vi "Ball Valve labVIEW Code.vi"() -> ()   [LabVIEW 2025]
uses:
  PIDController/PIDController.lvclass
  spikeController/spikeController.lvclass
  labjacksModeEnum.ctl
  ControllerModeEnum.ctl
  modesEnum.ctl
  PIDController/PIDController.lvclass/PIDController.ctl
  0285ecf2-4d18-4427-ace1-61b1951a0741.vi
  d3b0afdc-d7ac-4f1a-8ecc-0aeb21fe1e80.vi
  0890acf7-df83-934e-a7ac-ae51bc85d557.vi
  d872897a-af24-4a4d-87bc-a1bb59a840a8.vi
  <vilib>/Instr/_visa.llb/VISA Configure Serial Port (Instr).vi
  PIDController/updateLastValues.vi
  <vilib>/Utility/file.llb/Write Delimited Spreadsheet (string).vi
  <vilib>/Utility/file.llb/Write Delimited Spreadsheet (DBL).vi
  <vilib>/ptbypt/NI_PtbyPt.lvlib
panel:
  out "arduino read response":string
  out "start time":u32
  in  "timeout":dbl=300.0
  in  "direction":i32=1
  in  "bias":dbl=100.0
  out "auto state":i32
  out "auto \ncycle_count":i32
  out "elements":T1[](array[typedef])
  out "Current Sensor Mode":T1=enum."Connect to Labjack"
  out "Labjack Handle":i32
  in  "Sensor Mode":enum16{"Fake", "Redboard", "Labjacks"}(ring)
  in  "Connect arduino":bool
  out "Connected":bool
  out "Set Angle":cluster{"Value":dbl, "Value":dbl}(graph)
  out "Read angle":dbl
  out "Target Angle":dbl
  out "arduino status":bool
  out "Motor Response":string
  in  "Disconnect":bool
  in  "Start Program":bool
  in  "Use Dummy Data":bool
  out "Pressure Sensor (integrated)":dbl(graph)
  out "PID Raw (one-by-one)":dbl(graph)
  out "target PID point":dbl
  out "auto k_d":dbl
  out "auto k_i":dbl
  out "auto k_p":dbl
  out "Array-to-save":dbl[][](array[numeric])
  out "to save":path
  out "Time Elapsed":dbl
  out "cycles_run":i32
  out "Autotune":bool
  in  "dt":dbl=0.1
  in  "tuning_rule":i32=3
  in  "min_cycles":i32=4
  in  "hysteresis":dbl=0.5
  in  "relay_amplitude":dbl=10.0
  in  "Exit Autotune":bool
  in  "Start AutoTune":bool
  out "last error":dbl
  in  "Use D1":bool
  in  "Use D2":bool
  in  "Use Avg":bool
  in  "Save Graphs":bool
  in  "Set setPoint":dbl=100.0 format="%.3f"
  in  "Set Angle":dbl format="%.3f"
  in  "setPoint Dial":dbl(knob) scale=0.0..1000.0
  in  "A_max":dbl=180.0
  in  "A_min":dbl
  in  "k_i":dbl
  in  "k_d":dbl
  in  "k_p":dbl
  out "SafetyClose":bool
  out "PID":bool
  out "Manual":bool
  out "Idle":bool
  out "Ducer1":bool
  out "Ducer2":bool
  out "Avg Ducers":bool
  out "Read Pressure Ducer":dbl
  out "Pressure Ducer 2":dbl
  in  "spikeController.lvclass":refnum<class "spikeController.lvclass">
  out "underAmin":bool
  out "overAmax":bool
  out "PID Raw Output":dbl[](graph)
  out "PID Translated Output":dbl
  out "PID Raw Output":dbl
  in  "loop stop 2":bool
  in  "loop stop 1":bool
  in  "PIDController.lvclass":refnum<class "PIDController.lvclass">
  in  "?":u32(colorbox)=16777225
  out "Pressure Sensor":dbl[](graph)
  in  "motor rpm indicator":dbl
  out "Motor Signal":string
  in  "stop program":bool
  in  "return spike":bool
  out "Position (measured)":dbl[](graph)
  out "Arduino Error":errorcluster
  in  "VISA resource Port":refnum<visa-resource-name>
  out "distance to go":dbl caption="Rotations to Go (º)" format="%.3f"
  out "Current Angle":dbl format="%.3f"
  in  "Set Angle (º)":dbl(slide) scale=0.1..180.0
  out "?":dbl(slide) scale=0.0..1000.0
  out "Stagnation Flow Temp (K)":dbl
  out "Pressure Ducer":dbl
  in  "Sensor Offsets":dbl[](array[numeric])=[10.0, 10.0, 0.0, 22.0]
  in  "Sensor K-values":dbl[](array[numeric])=[10.0, 10.0, 0.0, 22.0]
  in  "Exit PID Mode":bool
  in  "manual exit button":bool
  in  "Motor Control Loop Rate (ms)":dbl
  out "Set Motor RPM":dbl(knob) scale=0.0..200.0
  in  "PID Mode":bool
  in  "Manual Positioning Mode":bool
  in  "Stop Sensors":bool
  in  "Sensor Loop Rate (ms)":dbl
  out "Time Since Start (s)\n(For Reference Only)":dbl format="%.2f"
  in  "Start Sensors":bool
  in  "Load Inputs":bool
  in  "Save Inputs":bool
  out "Port":i32
  out "ConnectionType":i32
  out "DeviceType":i32
  out "Labjack error":errorcluster
  # "(dial indicator for range)"
  # "34HS59-6004S Motor Torque Curve (For Reference)"
  # "Labjack/Arduino Resources"
  # "Inputs and LabJack Sensor Monitors"
  # "PID Inputs"
  # "Motor RPM >200 RPM"
  # "Potentiometer"
  # "Inefficent Torque for High Mass Flow/Thrust Tests"
  # "Ducer"
  # "<-- Uses same setpoint"
  # "Thermocouple"
  # "Motor RPM < 200 RPM"
  # "COM Port for Arduino"
  # "Ball valve"
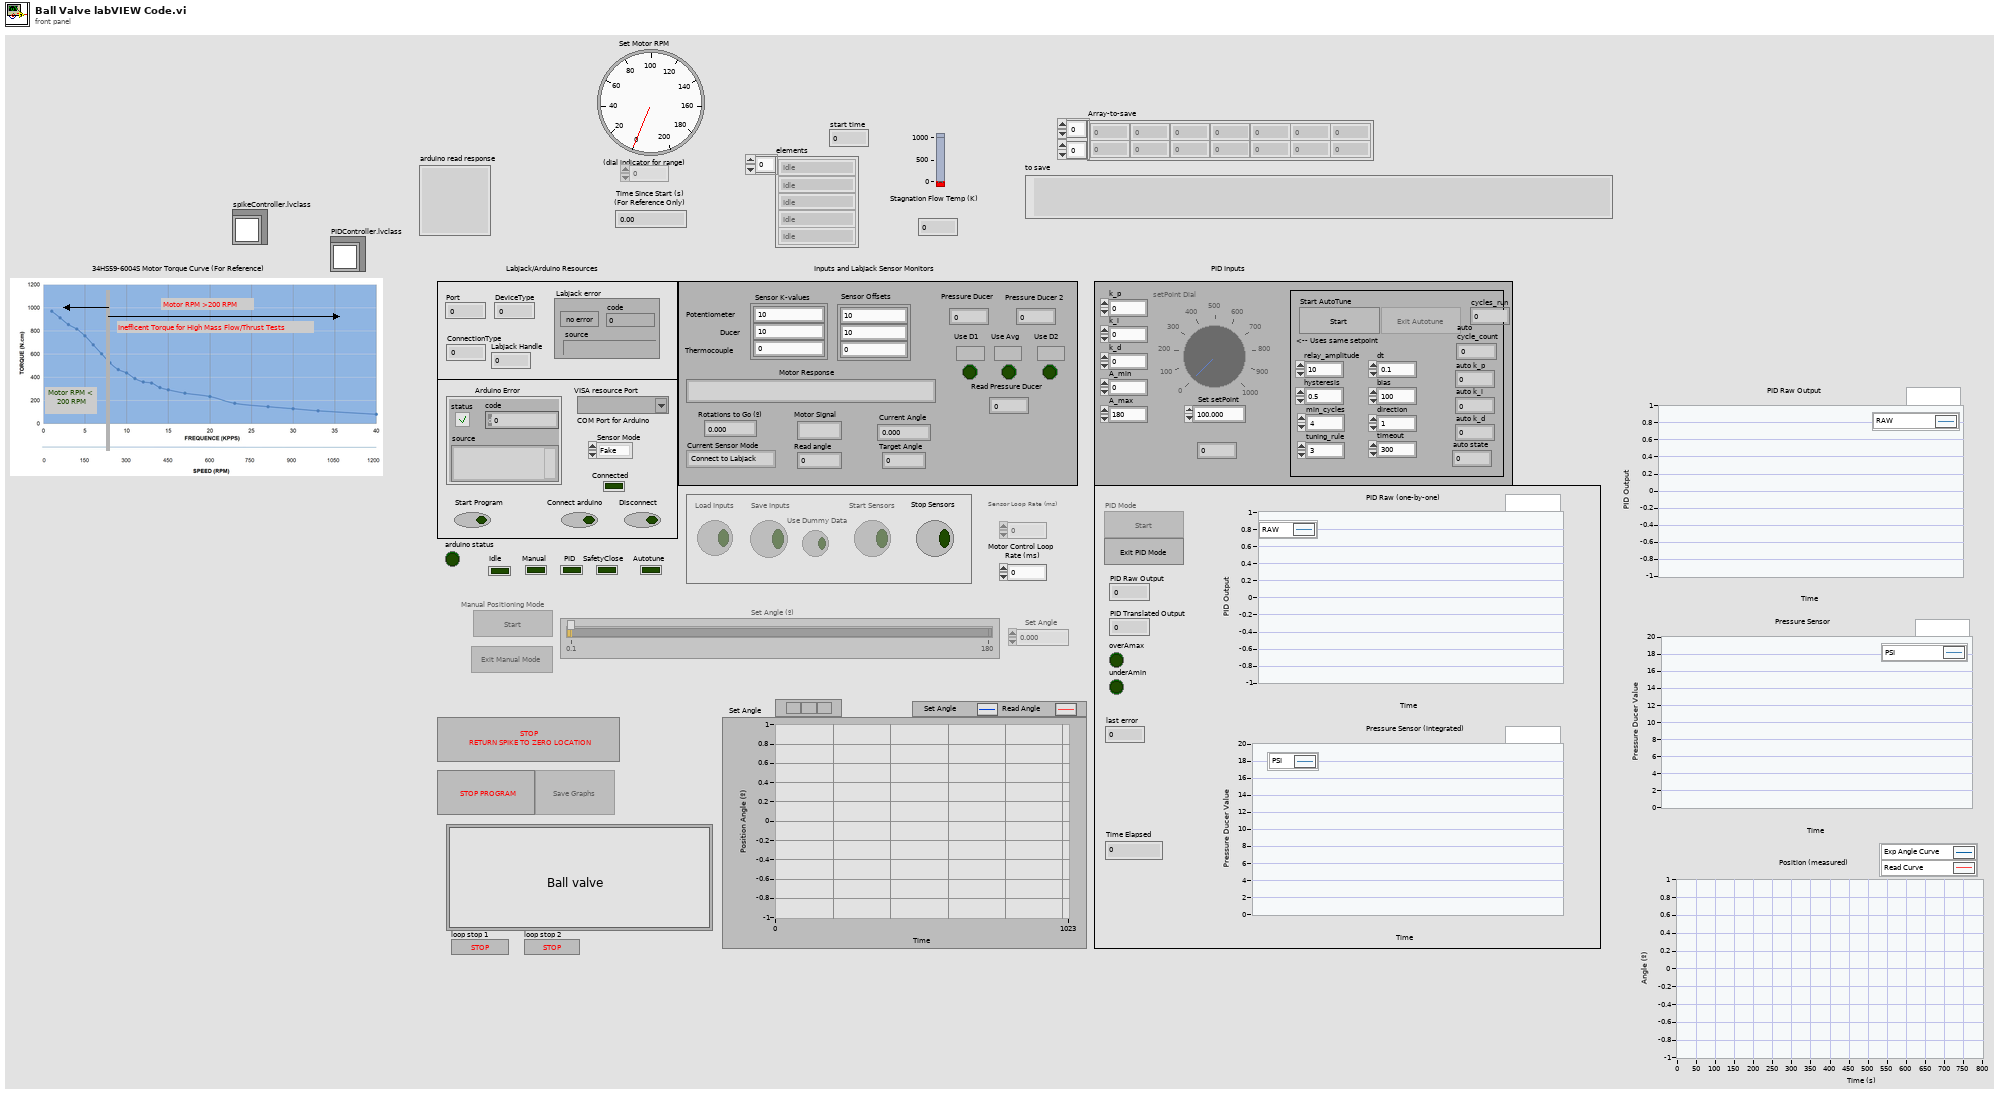
[diagram p1: front panel]
types:
  T1 = typedef "labjacksModeEnum.ctl" = enum16{"Idle", "Connect to Labjack", "Start sensors", "Dummy data", "Arduino Sensors", "load values"}
  T2 = typedef "ControllerModeEnum.ctl" = enum16{"", "startControllers", "IdleControllers"}
  T3 = typedef "modesEnum.ctl" = enum16{"relay_autotune", "SafetyOpen", "SafetyClose", "SaveFile", "PIDControl", "ManualControl", "Idle"}
  T4 = enum16{"Potentiometer", "Ducer", "Thermocouple", "Ducer2"}
  T5 = enum16{"Ducer", "Ducer2", "Thermocouple", "Potentiometer"}
  T6 = enum8{"Enabled", "Disabled", "Disabled and Grayed Out"}
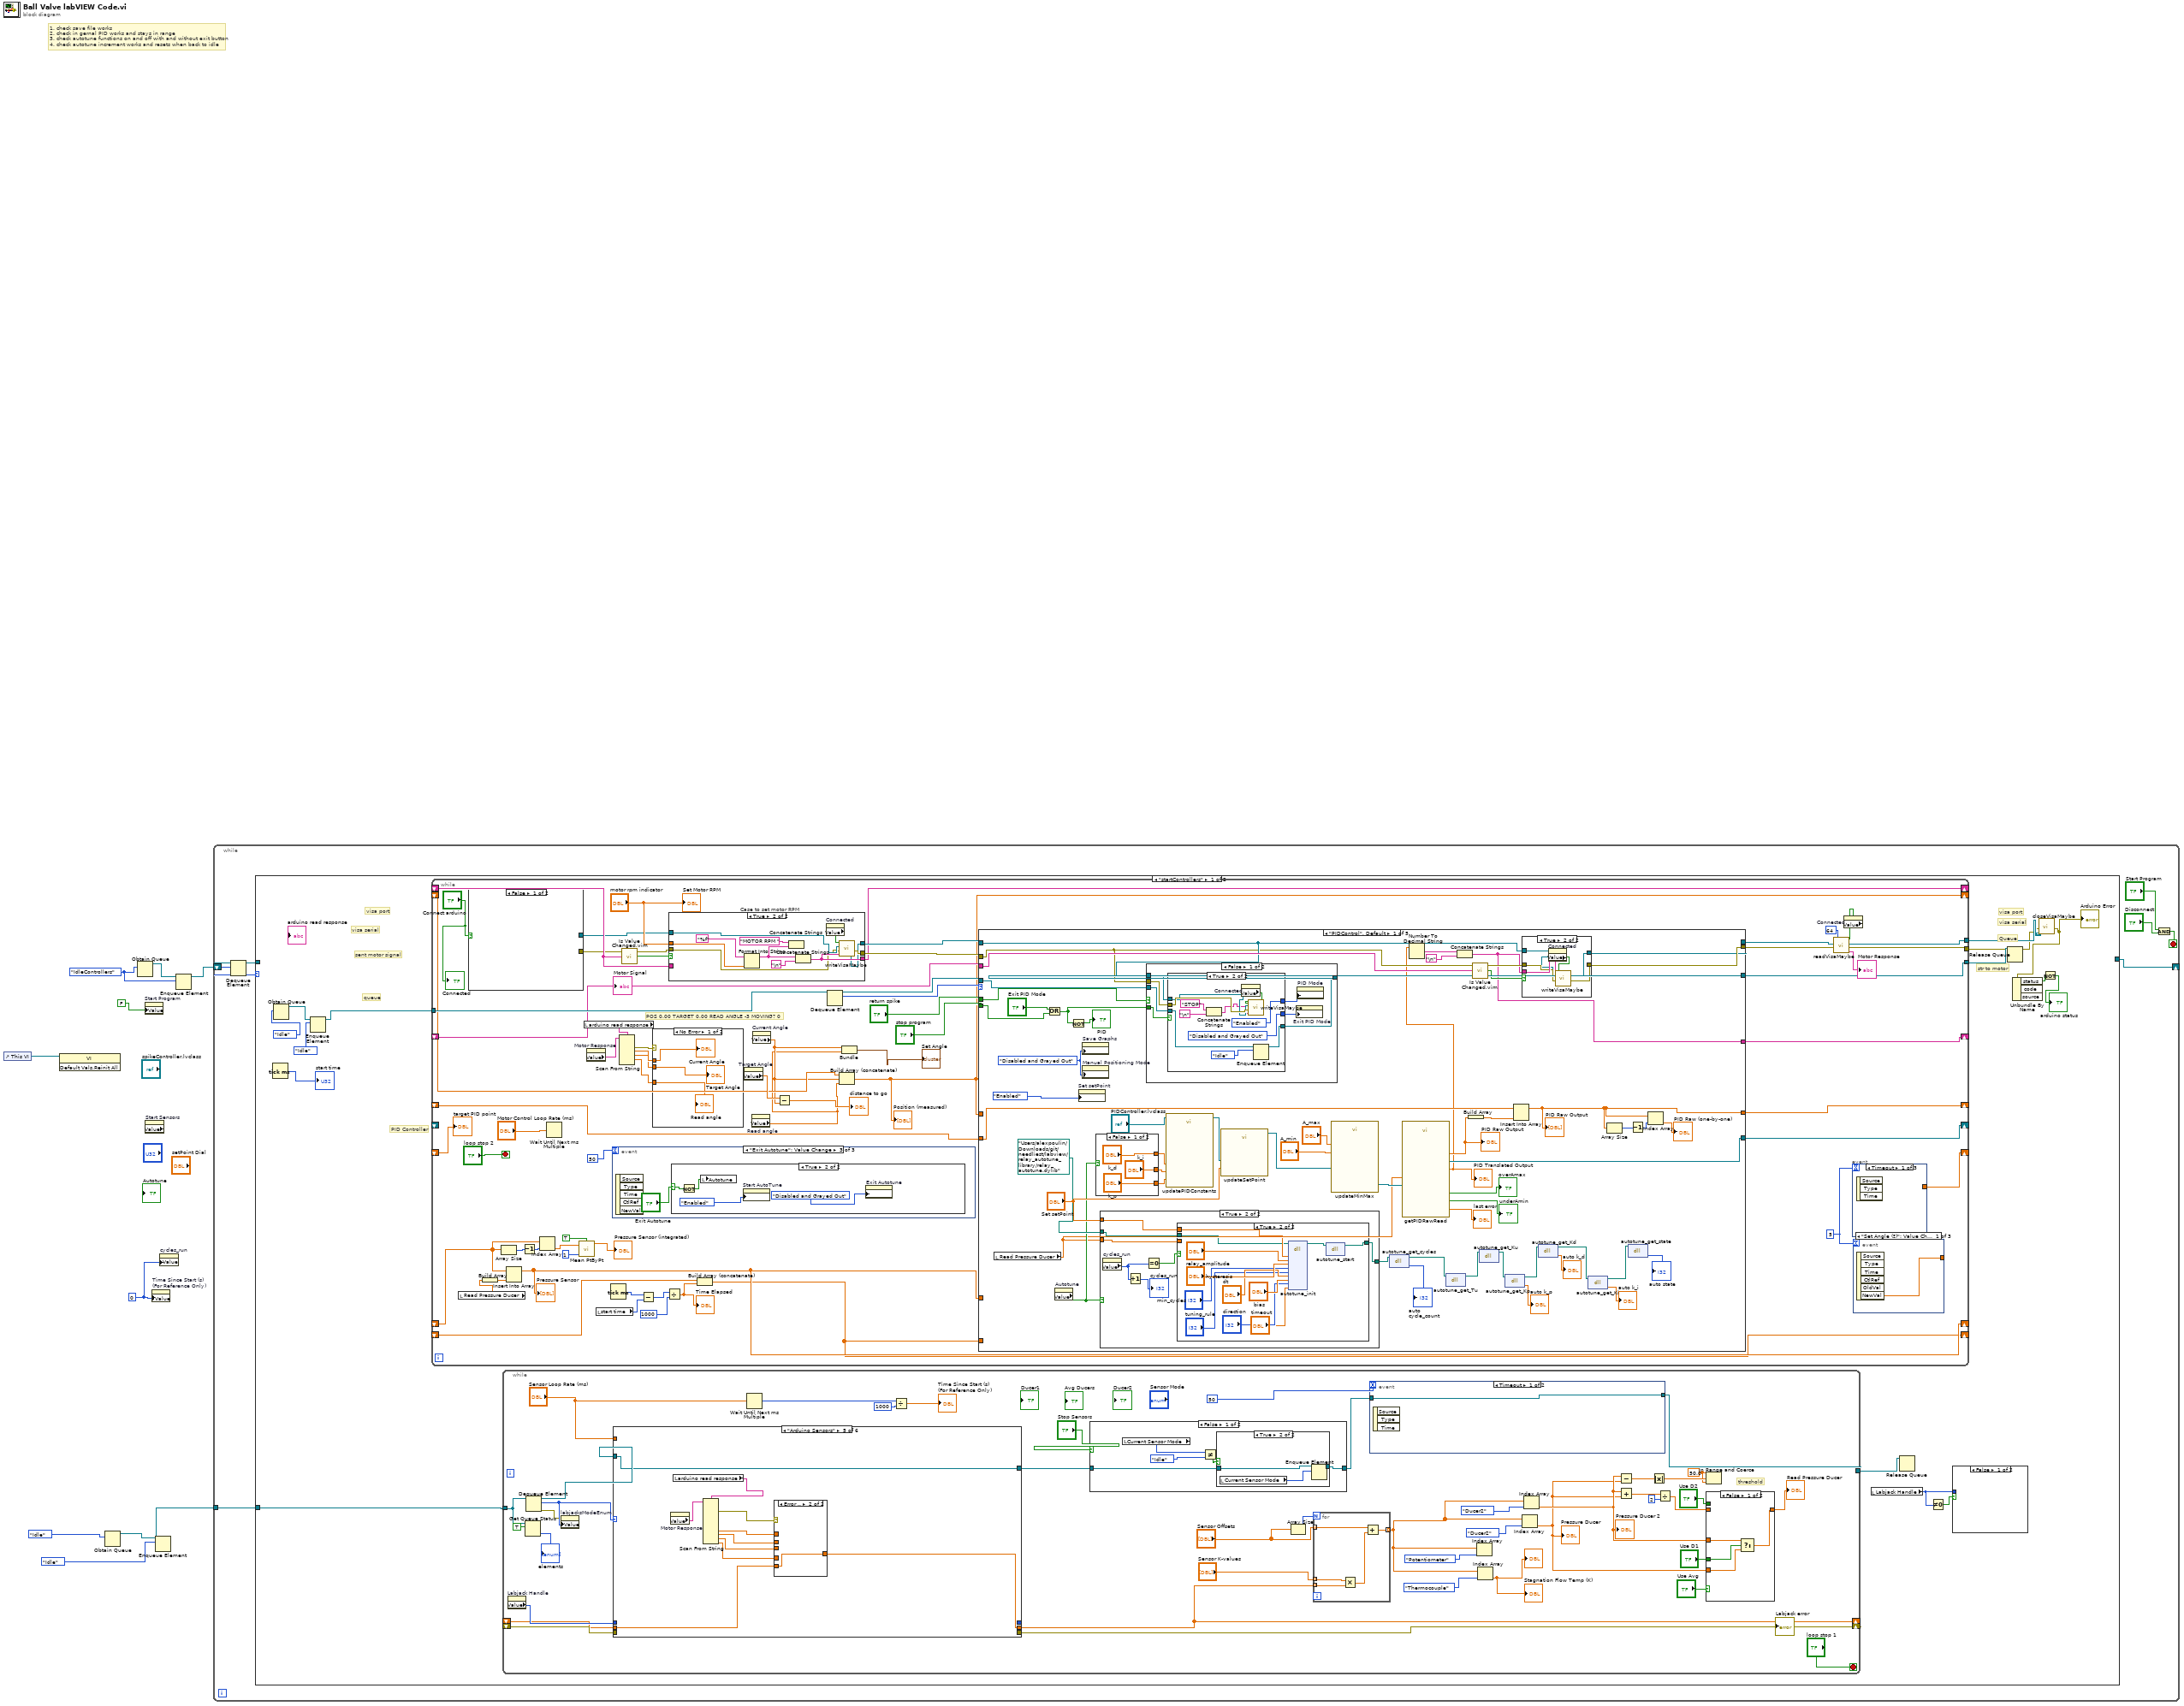
[diagram p0: block diagram]
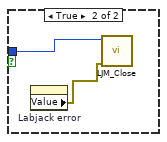
[diagram p2: hidden frame]
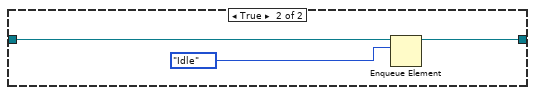
[diagram p4: hidden frame]
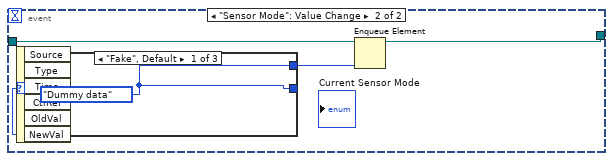
[diagram p5: hidden frame]
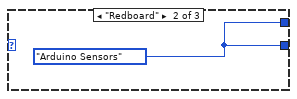
[diagram p6: hidden frame]
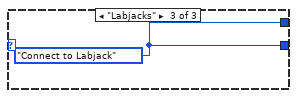
[diagram p7: hidden frame]
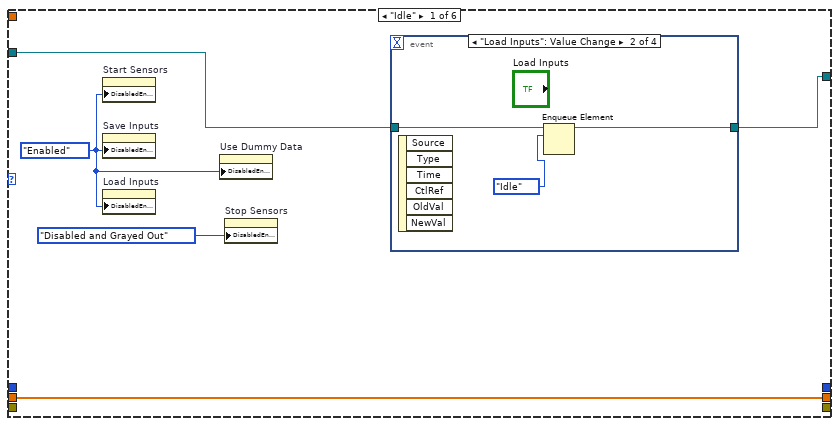
[diagram p9: hidden frame]
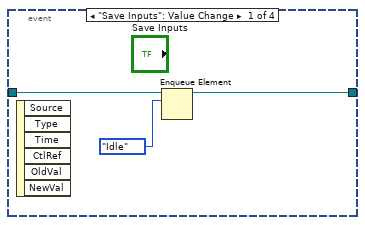
[diagram p10: hidden frame]
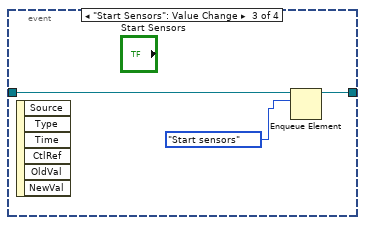
[diagram p11: hidden frame]
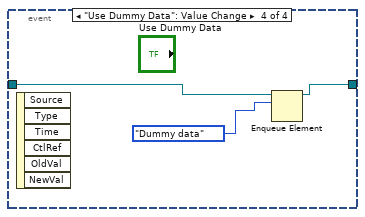
[diagram p12: hidden frame]
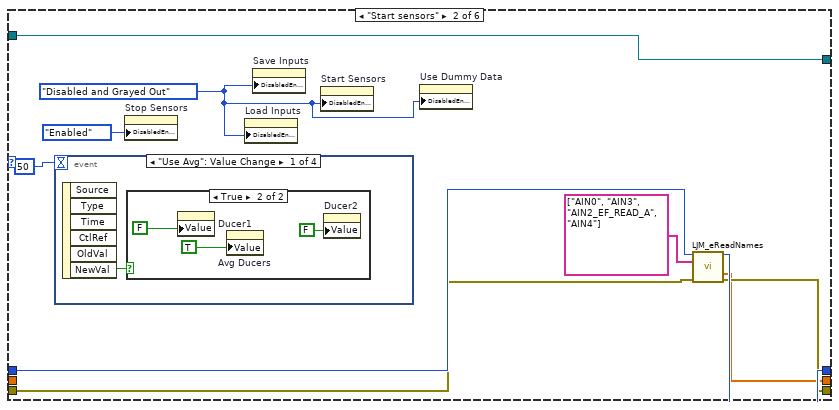
[diagram p13: hidden frame]
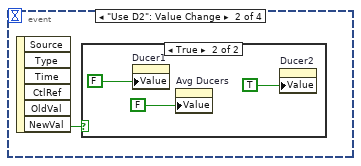
[diagram p15: hidden frame]
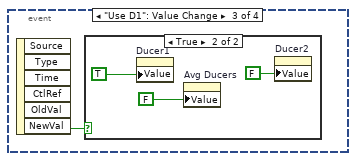
[diagram p17: hidden frame]
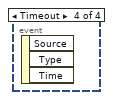
[diagram p19: hidden frame]
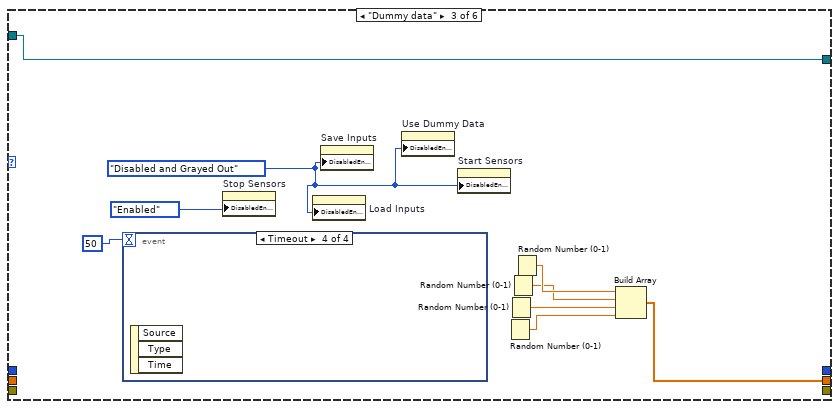
[diagram p20: hidden frame]
diagram:
  w2 = u32 0 ("Time Since Start (s)\n(For Reference Only) 2")
  w9 = ControllerModeEnum."IdleControllers" ("ControllerModeEnum")
  # "1. check save file works\n2. check in gernal PID works and stays in range\n3. check autotune functions on and off with and without exit button\n4. check autotune increment works and resets when back to idle"
  n1 = control-ref of="This VI"() -> (w1:refnum<vi>)
  n2 = invoke class="VI" method="Default Vals.Reinit All"(reference=w1) -> ()  [unwired: 2 in, 3 out]
  n3 = Obtain Queue(element data type=labjacksModeEnum."Idle" ("labjacksModeEnum")) -> (queue out=w5:refnum<queue>)  [unwired: 4 in, 2 out]
  n4 = Obtain Queue(element data type=w9) -> (queue out=w10:refnum<queue>)  [unwired: 4 in, 2 out]
  n5 = property on="Start Program" class="Bool (strict)"("Value"=FALSE) -> ()  [unwired: 2 in, 2 out]
  n6 = property on="Start Sensors" class="Bool" props=["Value"]() -> ()  [unwired: 2 in, 3 out]
  n7 = property on="Time Since Start (s)\n(For Reference Only)" class="DigNum (strict)"("Value"=w2) -> ()  [unwired: 2 in, 2 out]
  n8 = Enqueue Element(queue=w5, element=labjacksModeEnum."Idle" ("labjacksModeEnum")) -> (queue out=w3:refnum<queue>)  [unwired: 2 in, 2 out]
  n9 = property on="cycles_run" class="DigNum (strict)"("Value"=w2) -> ()  [unwired: 2 in, 2 out]
  n10 = Enqueue Element(queue=w10, element=w9) -> (queue out=w8:refnum<queue>)  [unwired: 2 in, 2 out]
  n11 = while {
    shift-right: [w14] -> _
    shift-left: w8 -> [w12]
    tunnel: w3 -> [w11]
    stop <- w16 stop-if-true
    n12 = Dequeue Element(queue=w12) -> (queue out=w13:refnum<queue>, element=w15:T2)  [unwired: 2 in, 2 out]
    n13 = case shown="\"startControllers\"" w15 {
      tunnel: [_ w568] -> w14
      tunnel: w13 -> [_ w567]
      tunnel: w11 -> [w22 _]
      frame "startControllers" {
        # "str to motor"
        # "Queue"
        # "sent motor signal"
        # "PID Controller"
        # "visa serial"
        # "visa port"
        # "queue"
        # "visa port"
        # "visa serial"
        n14 = Tick Count (ms)() -> (millisecond timer value=→"start time":u32)
        n15 = Obtain Queue(element data type=modesEnum."Idle" ("modesEnum")) -> (queue out=w33:refnum<queue>)  [unwired: 4 in, 2 out]
        n16 = Enqueue Element(queue=w33, element=modesEnum."Idle" ("modesEnum")) -> (queue out=w32:refnum<queue>)  [unwired: 2 in, 2 out]
        n17 = while {
          tunnel: w32 -> [w260]
          tunnel: [w258] -> w31
          tunnel: [w220] -> w26
          tunnel: [w221] -> w25
          shift-right: [w256] -> _
          shift-left: _ -> [w255]
          shift-right: [w251] -> _
          shift-left: _ -> [w250]
          shift-right: [w247] -> _
          shift-left: _ -> [_]
          shift-right: [w200] -> _
          shift-left: _ -> [w202]
          shift-right: [w244] -> _
          shift-left: _ -> [w245]
          shift-right: [w228] -> _
          shift-left: _ -> [w232]
          shift-right: [w240] -> _
          shift-left: _ -> [w241]
          shift-right: [w199] -> _
          shift-left: _ -> [w211]
          stop <- "loop stop 2" stop-if-true
          w239 = 5
          # "POS 0.00 TARGET 0.00 READ ANGLE -3 MOVING? 0"
          n18 = local read "Read Pressure Ducer"() -> (w201:dbl)
          n19 = case shown="False" "Connect arduino" {
            tunnel: [_ w271] -> w219
            tunnel: [_ w270] -> w218
            frame False {
            }
            frame True {
              w272 = u16 0 items=["None", "XON/XOFF", "RTS/CTS", "XON/XOFF & RTS/CTS", "DTR/DSR", "XON/XOFF & DTR/DSR"] ("flow control (0:none)")
              w273 = u16 10 items=["1.0"=10, "1.5"=15, "2.0"=20] ("stop bits (10: 1 bit)")
              n20 = call-poly "VISA Configure Serial Port"("VISA resource name"="VISA resource Port", "Enable Termination\nChar (T)"=TRUE ("Enable Termination\nChar (T)"), "baud rate (9600)"=u32 115200, "data bits (8)"=u16 8, "parity (0:none)"=enum16{"None", "Odd", "Even", "Mark", "Space"}."None", "stop bits (10: 1 bit)"=w273, "flow control (0:none)"=w272) -> ("VISA resource name out"=w271:refnum<visa-resource-name>, "error out"=w270:errorcluster)  [unwired: 7 in]
            }
          }
          n21 = Build Array(w201) -> (w205:dbl[])
          n22 = Array Size(array=w202) -> (size(s)=w208:i32)
          n23 = Insert Into Array(array=w202, new element=w205) -> (w200:dbl[])  [unwired: 1 in]
          "Pressure Sensor" <- w200
          n24 = Decrement(x=w208) -> (x-1=w209:i32)
          n25 = Index Array(array=w202, index=w209) -> (element=w206:dbl)
          n26 = Wait Until Next ms Multiple(millisecond multiple="Motor Control Loop Rate (ms)") -> ()  [unwired: 1 out]
          n27 = call <vilib>:"Mean PtByPt.vi"("x"=w206, "sample length"=1, "initialize"=TRUE) -> ("mean"=→"Pressure Sensor (integrated)":dbl)  [unwired: 1 in, 1 out]
          n28 = local read "arduino read response"() -> (w198:string)
          n29 = property on="Motor Response" class="Str"() -> ("Value"=w238:string)  [unwired: 2 in, 2 out]
          n30 = local read "start time"() -> (w215:u32)
          n31 = Tick Count (ms)() -> (millisecond timer value=w212:u32)
          n32 = event shown="[2] \"Exit Autotune\": Value Change" {
            selector: _ -> [_ _ _]
            dyn-events: _ -> [_ _ _]
            timeout: 50 -> [_ _ _]
            event Timeout {
              n33 = event-data() -> ()  [unwired: 1 in, 3 out]
            }
            event "Start AutoTune": Value Change {
              n34 = event-data() -> ()  [unwired: 1 in, 5 out]
              n35 = case shown="True" "Start AutoTune" {
                selector: "Start AutoTune" -> [w264 _]
                frame True {
                  n36 = local write "Autotune"(w264) -> ()
                  n37 = property on="Exit Autotune" class="Bool"("DisabledEnum"=T6."Enabled" ("Disabled")) -> ()  [unwired: 2 in, 2 out]
                  n38 = property on="Start AutoTune" class="Bool"("DisabledEnum"=T6."Disabled and Grayed Out" ("Disabled")) -> ()  [unwired: 2 in, 2 out]
                }
                frame False {
                }
              }
            }
            event "Exit Autotune": Value Change {
              n39 = event-data() -> ()  [unwired: 1 in, 5 out]
              n40 = case shown="True" "Exit Autotune" {
                selector: "Exit Autotune" -> [_ w269]
                frame False {
                }
                frame True {
                  n41 = Not(x=w269) -> (.not. x?=w266:bool)
                  n42 = local write "Autotune"(w266) -> ()
                  n43 = property on="Start AutoTune" class="Bool"("DisabledEnum"=T6."Enabled" ("Disabled")) -> ()  [unwired: 2 in, 2 out]
                  n44 = property on="Exit Autotune" class="Bool"("DisabledEnum"=T6."Disabled and Grayed Out" ("Disabled")) -> ()  [unwired: 2 in, 2 out]
                }
              }
            }
          }
          n45 = Scan From String(format string=w198, input string=w238) -> (error out=w237:errorcluster, output 1=w236:dbl, output 2=w234:dbl, output 3=w231:dbl)  [unwired: 7 in, 2 out]
          n46 = call "Is Value Changed.vim"("value"=w250) -> ("changed or first call?"=w252:bool)
          n47 = Subtract(x=w212, y=w215) -> (x-y=w214:u32)
          n48 = case shown="No Error" w237 {
            tunnel: w236 -> [w280 _]
            tunnel: w234 -> [w281 _]
            tunnel: w231 -> [w279 _]
            frame No Error {
              "Target Angle" <- w281
              "Current Angle" <- w280
              "Read angle" <- w279
            }
            frame Error {
            }
          }
          n49 = Divide(x=w214, y=1000) -> (x/y=w210:dbl)
          "Time Elapsed" <- w210
          n50 = case "Case to set motor RPM" shown="True" w252 {
            tunnel: w218 -> [w291 w296]
            tunnel: [w287 w298] -> w251
            tunnel: w219 -> [w292 w297]
            tunnel: [w291 w295] -> w254
            tunnel: [w292 w294] -> w253
            tunnel: "motor rpm indicator" -> [w290 w303]
            tunnel: w250 -> [_ _]
            frame False {
              n51 = Format Into String(format string="%f", w290) -> (resulting string=w288:string)  [unwired: 2 in, 1 out]
              n52 = Concatenate Strings(w288, "\n" ("string")) -> (w287:string)
            }
            frame True {
              n53 = Format Into String(format string="%f", w303) -> (resulting string=w301:string)  [unwired: 2 in, 1 out]
              n54 = Concatenate Strings("MOTOR RPM " ("format string"), w301) -> ()  [unwired: 1 out]
              n55 = Concatenate Strings(w301, "\n") -> (w298:string)
              n56 = property on="Connected" class="Bool (strict)"() -> ("Value"=w293:bool)  [unwired: 2 in, 2 out]
              n57 = call "writeVisaMaybe.vi"("String to Write"=w298, "error in"=w296, "VISA resource name in"=w297, "VISA connected?"=w293) -> ("error out"=w295:errorcluster, "VISA resource name out"=w294:refnum<visa-resource-name>)  [unwired: 2 in]
            }
          }
          n58 = Build Array (concatenate)(w211, w210) -> (w199:dbl[])
          n59 = property on="Target Angle" class="DigNum (strict)"() -> ("Value"=w233:dbl)  [unwired: 2 in, 2 out]
          n60 = property on="Read angle" class="DigNum (strict)"() -> ("Value"=w229:dbl)  [unwired: 2 in, 2 out]
          n61 = property on="Current Angle" class="DigNum (strict)"() -> ("Value"=w230:dbl)  [unwired: 2 in, 2 out]
          n62 = Subtract(x=w233, y=w230) -> (x-y=→"distance to go":dbl)
          n63 = Dequeue Element(queue=w260) -> (queue out=w242:refnum<queue>, element=w259:T3)  [unwired: 2 in, 2 out]
          n64 = Build Array (concatenate)(w232, w230, w229) -> (w228:dbl[])
          "Position (measured)" <- w228
          n65 = Bundle("Value"=w230, "Value"=w229) -> (→"Set Angle":cluster{"Value":dbl, "Value":dbl})  [unwired: 1 in]
          n66 = case shown="\"PIDControl\", Default" w259 {
            tunnel: [w351 w436 w473 w506 _] -> w258
            tunnel: w242 -> [w327 w432 w474 w505 _]
            tunnel: w253 -> [w326 w423 w471 w509 _]
            tunnel: [w315 w422 w470 w501 _] -> w226
            tunnel: w254 -> [w314 w425 w469 w510 _]
            tunnel: [w316 w421 w468 w507 _] -> w224
            tunnel: [w313 w424 w478 w508 _] -> w256
            tunnel: w255 -> [w347 _ w478 w504 _]
            tunnel: "return spike" -> [w350 w437 _ _ _]
            tunnel: [w358 _ _ _ _] -> w247
            tunnel: w245 -> [w320 _ _ _ w551]
            tunnel: [w312 _ _ _ _] -> w244
            tunnel: "stop program" -> [w352 w428 _ _ _]
            tunnel: w228 -> [_ _ _ _ w553]
            tunnel: w200 -> [_ _ _ _ w550]
            tunnel: w199 -> [_ _ _ _ w552]
            frame "PIDControl", Default {
              w330 = T6."Disabled and Grayed Out" ("Disabled")
              n67 = local read "Read Pressure Ducer"() -> (w304:dbl)
              n68 = Or(x="Exit PID Mode", y=w352) -> (x .or. y?=w328:bool)
              n69 = property on="Autotune" class="Bool (strict)"() -> ("Value"=w305:bool)  [unwired: 2 in, 2 out]
              n70 = Not(x=w328) -> (.not. x?=→"PID":bool)
              n71 = property on="Set setPoint" class="DigNum (strict)"("DisabledEnum"=T6."Enabled" ("Disabled")) -> ()  [unwired: 2 in, 2 out]
              n72 = property on="Save Graphs" class="Bool"("DisabledEnum"=w330) -> ()  [unwired: 2 in, 2 out]
              n73 = property on="Manual Positioning Mode" class="Bool"("DisabledEnum"=w330) -> ()  [unwired: 2 in, 2 out]
              n74 = case shown="False" w305 {
                tunnel: ["k_p" w362] -> w339
                tunnel: ["k_i" w363] -> w338
                tunnel: ["k_d" w364] -> w337
                frame False {
                }
                frame True {
                  n75 = local read "auto k_i"() -> (w363:dbl)
                  n76 = local read "auto k_d"() -> (w364:dbl)
                  n77 = local read "auto k_p"() -> (w362:dbl)
                }
              }
              n78 = case shown="True" w305 {
                tunnel: path "/Users/alexpoulin/Downloads/git/needliest/labview/relay_autotune_library/relay_autotune.dylib" -> [w371 w376]
                tunnel: [w371 w375] -> w340
                tunnel: w304 -> [_ w374]
                tunnel: "Set setPoint" -> [_ w372]
                frame False {
                }
                frame True {
                  n79 = property on="cycles_run" class="DigNum (strict)"() -> ("Value"=w378:i32)  [unwired: 2 in, 2 out]
                  n80 = Increment(x=w378) -> (x+1=→"cycles_run":i32)
                  n81 = Equal To 0?(x=w378) -> (x = 0?=w373:bool)
                  n82 = case shown="True" w373 {
                    tunnel: w376 -> [w381 w385]
                    tunnel: [w380 w392] -> w375
                    tunnel: w374 -> [w379 _]
                    tunnel: w372 -> [_ w386]
                    frame False {
                      n83 = dll-call lib="Users/alexpoulin/Downloads/git/needliest/labview/relay_autotune_library/relay_autotune.dylib" fn="autotune_update"(path in=w381, "pv"=w379) -> (path out=w380:path)  [unwired: 4 in, 1 out]
                    }
                    frame True {
                      n84 = dll-call lib="Users/alexpoulin/Downloads/git/needliest/labview/relay_autotune_library/relay_autotune.dylib" fn="autotune_init"(path in=w385, "setpoint"=w386, "relay_amplitude"="relay_amplitude", "hysteresis"="hysteresis", "min_cycles"="min_cycles", "tuning_rule"="tuning_rule", "dt"="dt", "bias"="bias", "direction"="direction", "timeout"="timeout") -> (path out=w393:path)  [unwired: 12 in, 1 out]
                      n85 = dll-call lib="Users/alexpoulin/Downloads/git/needliest/labview/relay_autotune_library/relay_autotune.dylib" fn="autotune_start"(path in=w393) -> (path out=w392:path)  [unwired: 3 in, 1 out]
                    }
                  }
                }
              }
              n86 = case shown="False" w350 {
                tunnel: [w396 w419] -> w351
                tunnel: w328 -> [w400 _]
                tunnel: w327 -> [w399 w417]
                tunnel: w326 -> [w398 _]
                tunnel: w314 -> [w397 _]
                frame False {
                  n87 = case shown="True" w400 {
                    tunnel: w399 -> [w405 w416]
                    tunnel: [w404 w415] -> w396
                    tunnel: w398 -> [_ w407]
                    tunnel: w397 -> [_ w408]
                    tunnel: [T6."Disabled and Grayed Out" ("Disabled") T6."Enabled" ("Disabled")] -> w395
                    tunnel: [T6."Enabled" ("Disabled") T6."Disabled and Grayed Out" ("Disabled")] -> w394
                    frame False {
                      n88 = Enqueue Element(queue=w405, element=modesEnum."PIDControl" ("modesEnum")) -> (queue out=w404:refnum<queue>)  [unwired: 2 in, 2 out]
                    }
                    frame True {
                      n89 = Concatenate Strings("STOP" ("write buffer"), "\n" ("write buffer")) -> (w406:string)
                      n90 = property on="Connected" class="Bool (strict)"() -> ("Value"=w409:bool)  [unwired: 2 in, 2 out]
                      n91 = call "writeVisaMaybe.vi"("String to Write"=w406, "error in"=w408, "VISA resource name in"=w407, "VISA connected?"=w409) -> ()  [unwired: 2 in, 2 out]
                      n92 = Enqueue Element(queue=w416, element=modesEnum."Idle" ("modesEnum")) -> (queue out=w415:refnum<queue>)  [unwired: 2 in, 2 out]
                    }
                  }
                  n93 = property on="Exit PID Mode" class="Bool"("DisabledEnum"=w394) -> ()  [unwired: 2 in, 2 out]
                  n94 = property on="PID Mode" class="Bool"("DisabledEnum"=w395) -> ()  [unwired: 2 in, 2 out]
                }
                frame True {
                  n95 = Enqueue Element(queue=w417, element=modesEnum."SafetyClose" ("modesEnum")) -> (queue out=w419:refnum<queue>)  [unwired: 2 in, 2 out]
                }
              }
              n96 = call "updatePIDConstants.vi"("new k_d"=w337, "new k_p"=w339, "new k_i"=w338, "PIDController in"="PIDController.lvclass") -> ("PIDController out"=w333:refnum<class "PIDController.lvclass">)  [unwired: 6 in, 1 out]
              n97 = call "updateSetPoint.vi"("new setpoint"="Set setPoint", "PIDController in"=w333) -> ("PIDController out"=w332:refnum<class "PIDController.lvclass">)  [unwired: 8 in, 1 out]
              n98 = call "updateMinMax.vi"("a_max"="A_max", "a_min"="A_min", "PIDController in"=w332) -> ("PIDController out"=w331:refnum<class "PIDController.lvclass">)  [unwired: 7 in, 1 out]
              n99 = dll-call lib="Users/alexpoulin/Downloads/git/needliest/labview/relay_autotune_library/relay_autotune.dylib" fn="autotune_get_cycles"(path in=w340) -> (path out=w346:path, "g_ctx.cycle_count"=→"auto \ncycle_count":i32)  [unwired: 2 in, 1 out]
              n100 = call "getPIDRawRead.vi"("sensorValue"=w304, "PIDController in"=w331) -> ("overAmin"=→"underAmin":bool, "translatedPIDOutput"=w309:dbl, "PIDRawRead"=w357:dbl, "PIDController out"=w358:refnum<class "PIDController.lvclass">, "underAmax"=→"overAmax":bool, "lastErrorRead"=→"last error":dbl)  [unwired: 4 in]
              "PID Raw Output" <- w357
              "PID Translated Output" <- w309
              n101 = Number To Decimal String(number=w309) -> (decimal integer string=w310:string)  [unwired: 1 in]
              n102 = dll-call lib="Users/alexpoulin/Downloads/git/needliest/labview/relay_autotune_library/relay_autotune.dylib" fn="autotune_get_Tu"(path in=w346) -> (path out=w345:path)  [unwired: 3 in, 1 out]
              n103 = Concatenate Strings(w310, "\n") -> (w313:string)
              n104 = Build Array(w357) -> (w356:dbl[])
              n105 = call "Is Value Changed.vim"("value"=w347) -> ("changed or first call?"=w317:bool)
              n106 = dll-call lib="Users/alexpoulin/Downloads/git/needliest/labview/relay_autotune_library/relay_autotune.dylib" fn="autotune_get_Ku"(path in=w345) -> (path out=w344:path)  [unwired: 3 in, 1 out]
              n107 = dll-call lib="Users/alexpoulin/Downloads/git/needliest/labview/relay_autotune_library/relay_autotune.dylib" fn="autotune_get_Kp"(path in=w344) -> (path out=w343:path, "g_ctx.Kp"=→"auto k_p":dbl)  [unwired: 2 in, 1 out]
              n108 = Insert Into Array(array=w320, new element=w356) -> (w312:dbl[])  [unwired: 1 in]
              "PID Raw Output" <- w312
              n109 = case shown="True" w317 {
                tunnel: w314 -> [_ w369]
                tunnel: w326 -> [_ w368]
                tunnel: [_ w367] -> w316
                tunnel: [_ w366] -> w315
                tunnel: w313 -> [_ w370]
                frame False {
                }
                frame True {
                  n110 = property on="Connected" class="Bool (strict)"() -> ("Value"=w365:bool)  [unwired: 2 in, 2 out]
                  n111 = call "writeVisaMaybe.vi"("String to Write"=w370, "error in"=w369, "VISA resource name in"=w368, "VISA connected?"=w365) -> ("error out"=w367:errorcluster, "VISA resource name out"=w366:refnum<visa-resource-name>)  [unwired: 2 in]
                }
              }
              n112 = dll-call lib="Users/alexpoulin/Downloads/git/needliest/labview/relay_autotune_library/relay_autotune.dylib" fn="autotune_get_Kd"(path in=w343) -> (path out=w342:path, "g_ctx.Kd"=→"auto k_d":dbl)  [unwired: 2 in, 1 out]
              n113 = dll-call lib="Users/alexpoulin/Downloads/git/needliest/labview/relay_autotune_library/relay_autotune.dylib" fn="autotune_get_Ki"(path in=w342) -> (path out=w341:path, "g_ctx.Ki"=→"auto k_i":dbl)  [unwired: 2 in, 1 out]
              n114 = Array Size(array=w312) -> (size(s)=w319:i32)
              n115 = dll-call lib="Users/alexpoulin/Downloads/git/needliest/labview/relay_autotune_library/relay_autotune.dylib" fn="autotune_get_state"(path in=w341) -> ("g_ctx.state"=→"auto state":i32)  [unwired: 2 in, 2 out]
              n116 = Decrement(x=w319) -> (x-1=w318:i32)
              n117 = Index Array(array=w312, index=w318) -> (element=→"PID Raw (one-by-one)":dbl)
            }
            frame "ManualControl" {
              w431 = T6."Enabled" ("Disabled")
              w434 = T6."Disabled and Grayed Out" ("Disabled")
              n118 = Or(x=w428, y="manual exit button") -> (x .or. y?=w438:bool)
              n119 = Or(x=w437, y=w438) -> (x .or. y?=w433:bool)
              n120 = Not(x=w433) -> (.not. x?=→"Manual":bool)
              n121 = case shown="False" w437 {
                tunnel: [w441 w464] -> w436
                tunnel: w433 -> [w445 _]
                tunnel: w432 -> [w444 w462]
                tunnel: w423 -> [w443 _]
                tunnel: w425 -> [w442 _]
                frame False {
                  n122 = case shown="True" w445 {
                    tunnel: w444 -> [w450 w461]
                    tunnel: [w449 w460] -> w441
                    tunnel: w443 -> [_ w452]
                    tunnel: w442 -> [_ w453]
                    tunnel: [T6."Enabled" ("Disabled") T6."Disabled and Grayed Out" ("Disabled")] -> w440
                    tunnel: [T6."Disabled and Grayed Out" ("Disabled") T6."Enabled" ("Disabled")] -> w439
                    frame False {
                      n123 = Enqueue Element(queue=w450, element=modesEnum."ManualControl" ("modesEnum")) -> (queue out=w449:refnum<queue>)  [unwired: 2 in, 2 out]
                    }
                    frame True {
                      n124 = Concatenate Strings("STOP" ("write buffer"), "\n") -> (w451:string)
                      n125 = property on="Connected" class="Bool (strict)"() -> ("Value"=w454:bool)  [unwired: 2 in, 2 out]
                      n126 = call "writeVisaMaybe.vi"("String to Write"=w451, "error in"=w453, "VISA resource name in"=w452, "VISA connected?"=w454) -> ()  [unwired: 2 in, 2 out]
                      n127 = Enqueue Element(queue=w461, element=modesEnum."Idle" ("modesEnum")) -> (queue out=w460:refnum<queue>)  [unwired: 2 in, 2 out]
                    }
                  }
                  n128 = property on="Manual Positioning Mode" class="Bool"("DisabledEnum"=w439) -> ()  [unwired: 2 in, 2 out]
                  n129 = property on="Manual Exit state" class="Bool"("DisabledEnum"=w440) -> ()  [unwired: 2 in, 2 out]
                }
                frame True {
                  n130 = Enqueue Element(queue=w462, element=modesEnum."SafetyClose" ("modesEnum")) -> (queue out=w464:refnum<queue>)  [unwired: 2 in, 2 out]
                }
              }
              n131 = property on="Set Angle (º)" class="Slide (strict)"("DisabledEnum"=w431) -> ()  [unwired: 2 in, 2 out]
              n132 = property on="Set Angle" class="DigNum (strict)"("DisabledEnum"=w431) -> ()  [unwired: 2 in, 2 out]
              n133 = property on="PID Mode" class="Bool"("DisabledEnum"=w434) -> ()  [unwired: 2 in, 2 out]
              n134 = property on="Save Graphs" class="Bool"("DisabledEnum"=w434) -> ()  [unwired: 2 in, 2 out]
              n135 = property on="Start AutoTune" class="Bool"("DisabledEnum"=w434) -> ()  [unwired: 2 in, 2 out]
              n136 = Number To Decimal String(number="Set Angle (º)") -> (decimal integer string=w430:string)  [unwired: 1 in]
              n137 = Concatenate Strings(w430, "\n") -> (w424:string)
              n138 = property on="Connected" class="Bool (strict)"() -> ("Value"=w420:bool)  [unwired: 2 in, 2 out]
              n139 = call "writeVisaMaybe.vi"("String to Write"=w424, "error in"=w425, "VISA resource name in"=w423, "VISA connected?"=w420) -> ("error out"=w421:errorcluster, "VISA resource name out"=w422:refnum<visa-resource-name>)  [unwired: 2 in]
            }
            frame "Idle" {
              w472 = T6."Disabled and Grayed Out" ("Disabled")
              w465 = T6."Disabled and Grayed Out" ("Disabled")
              w477 = T6."Enabled" ("Disabled")
              n140 = property on="SafetyClose" class="Bool (strict)"("Value"=FALSE) -> ()  [unwired: 2 in, 2 out]
              n141 = event shown="[2] \"Save Graphs\": Value Change" {
                selector: _ -> [_ _ _ _ _]
                dyn-events: _ -> [_ _ _ _ _]
                timeout: 50 -> [_ _ _ _ _]
                tunnel: w474 -> [w484 w487 w491 w495 w496]
                tunnel: [w483 w486 w490 w494 w497] -> w473
                tunnel: [_ TRUE _ _ _] -> w466
                event "Manual Positioning Mode": Value Change {
                  n142 = event-data() -> ()  [unwired: 1 in, 6 out]
                  n143 = Enqueue Element(queue=w484, element=modesEnum."ManualControl" ("modesEnum")) -> (queue out=w483:refnum<queue>)  [unwired: 2 in, 2 out]
                }
                event Timeout {
                  n144 = event-data() -> ()  [unwired: 1 in, 3 out]
                  n145 = Enqueue Element(queue=w487, element=modesEnum."Idle" ("modesEnum")) -> (queue out=w486:refnum<queue>)  [unwired: 2 in, 2 out]
                }
                event "Save Graphs": Value Change {
                  n146 = event-data() -> ()  [unwired: 1 in, 6 out]
                  n147 = Enqueue Element(queue=w491, element=modesEnum."SaveFile" ("modesEnum")) -> (queue out=w490:refnum<queue>)  [unwired: 2 in, 2 out]
                }
                event "PID Mode": Value Change {
                  n148 = event-data() -> ()  [unwired: 1 in, 6 out]
                  n149 = Enqueue Element(queue=w495, element=modesEnum."PIDControl" ("modesEnum")) -> (queue out=w494:refnum<queue>)  [unwired: 2 in, 2 out]
                  n150 = property on="Start AutoTune" class="Bool"("DisabledEnum"=T6."Enabled" ("Disabled")) -> ()  [unwired: 2 in, 2 out]
                }
                event "return spike": Value Change {
                  n151 = event-data() -> ()  [unwired: 1 in, 6 out]
                  n152 = Enqueue Element(queue=w496, element=modesEnum."SafetyClose" ("modesEnum")) -> (queue out=w497:refnum<queue>)  [unwired: 2 in, 2 out]
                }
              }
              "Idle" <- w466
              n153 = property on="Idle" class="Bool (strict)"("Value"=TRUE) -> ()  [unwired: 2 in, 2 out]
              n154 = Concatenate Strings("STOP" ("write buffer"), "\n" ("write buffer")) -> (w481:string)
              n155 = property on="Save Graphs" class="Bool"("DisabledEnum"=w477) -> ()  [unwired: 2 in, 2 out]
              n156 = property on="Manual Positioning Mode" class="Bool"("DisabledEnum"=w477) -> ()  [unwired: 2 in, 2 out]
              n157 = property on="PID Mode" class="Bool"("DisabledEnum"=w477) -> ()  [unwired: 2 in, 2 out]
              n158 = VISA Write(VISA resource name=w471, write buffer=w481, error in (no error)=w469) -> (VISA resource name out=w470:refnum<visa-resource-name>, error out=w468:errorcluster)  [unwired: 1 out]
              n159 = property on="Start AutoTune" class="Bool"("DisabledEnum"=w465) -> ()  [unwired: 2 in, 2 out]
              n160 = property on="Set setPoint" class="DigNum (strict)"("DisabledEnum"=w472) -> ()  [unwired: 2 in, 2 out]
              n161 = property on="Set Angle" class="DigNum (strict)"("DisabledEnum"=w472) -> ()  [unwired: 2 in, 2 out]
              n162 = property on="Set Angle (º)" class="Slide (strict)"("DisabledEnum"=w472) -> ()  [unwired: 2 in, 2 out]
              n163 = property on="Exit Autotune" class="Bool"("DisabledEnum"=w472) -> ()  [unwired: 2 in, 2 out]
              n164 = property on="PID Exit" class="Bool"("DisabledEnum"=w465) -> ()  [unwired: 2 in, 2 out]
              n165 = property on="Manual Exit" class="Bool"("DisabledEnum"=w465) -> ()  [unwired: 2 in, 2 out]
            }
            frame "SafetyClose" {
              w503 = T6."Disabled and Grayed Out" ("Disabled")
              # "Motor Signaling Structure"
              n166 = property on="Current Angle" class="DigNum (strict)"() -> ("Value"=w500:dbl)  [unwired: 2 in, 2 out]
              n167 = Equal To 0?(x=w500) -> (x = 0?=w499:bool)
              n168 = case shown="True" w499 {
                tunnel: w509 -> [w518 w536]
                tunnel: [w516 w533] -> w501
                tunnel: w510 -> [w519 w532]
                tunnel: [w517 w531] -> w507
                tunnel: [w511 w528] -> w508
                tunnel: w504 -> [w515 w535]
                tunnel: w505 -> [_ w527]
                tunnel: [_ w526] -> w506
                frame False {
                  n169 = call "Is Value Changed.vim"("value"=w515) -> ("changed or first call?"=w514:bool)
                  n170 = Concatenate Strings("0" ("write buffer"), "\n" ("write buffer")) -> (w511:string)
                  n171 = case shown="True" w514 {
                    tunnel: w519 -> [_ w524]
                    tunnel: w518 -> [_ w523]
                    tunnel: [_ w522] -> w517
                    tunnel: [_ w521] -> w516
                    tunnel: w511 -> [_ w520]
                    frame False {
                    }
                    frame True {
                      n172 = VISA Write(VISA resource name=w523, write buffer=w520, error in (no error)=w524) -> (VISA resource name out=w521:refnum<visa-resource-name>, error out=w522:errorcluster)  [unwired: 1 out]
                    }
                  }
                }
                frame True {
                  n173 = call "Is Value Changed.vim"("value"=w535) -> ("changed or first call?"=w534:bool)
                  n174 = Enqueue Element(queue=w527, element=modesEnum."Idle" ("modesEnum")) -> (queue out=w526:refnum<queue>)  [unwired: 2 in, 2 out]
                  n175 = Concatenate Strings("STOP" ("write buffer"), "\n" ("write buffer")) -> (w528:string)
                  n176 = case shown="True" w534 {
                    tunnel: w528 -> [_ w541]
                    tunnel: w536 -> [_ w540]
                    tunnel: [_ w539] -> w533
                    tunnel: w532 -> [_ w538]
                    tunnel: [_ w537] -> w531
                    frame False {
                    }
                    frame True {
                      n177 = VISA Write(VISA resource name=w540, write buffer=w541, error in (no error)=w538) -> (VISA resource name out=w539:refnum<visa-resource-name>, error out=w537:errorcluster)  [unwired: 1 out]
                    }
                  }
                }
              }
              n178 = property on="Exit PID Mode" class="Bool"("DisabledEnum"=w503) -> ()  [unwired: 2 in, 2 out]
              n179 = property on="PID Mode" class="Bool"("DisabledEnum"=w503) -> ()  [unwired: 2 in, 2 out]
              n180 = property on="Manual Positioning Mode" class="Bool"("DisabledEnum"=w503) -> ()  [unwired: 2 in, 2 out]
              n181 = property on="manual exit button" class="Bool"("DisabledEnum"=w503) -> ()  [unwired: 2 in, 2 out]
              n182 = property on="Start AutoTune" class="Bool"("DisabledEnum"=w503) -> ()  [unwired: 2 in, 2 out]
              "SafetyClose" <- TRUE
            }
            frame "SaveFile" {
              w545 = ","
              n183 = Get Date/Time In Seconds() -> (seconds since 1Jan1904=w562:timestamp)
              n184 = Seconds To Date/Time(time stamp (now)=w562) -> ()  [unwired: 1 in, 1 out]
              n185 = Format Date/Time String(time format string (%c)="%Y-%m-%d_%H-%M-%S", seconds (now)=w562) -> (date/time string=w564:string)  [unwired: 1 in]
              n186 = Concatenate Strings("/needleValveData_", w564) -> (w557:string)
              n187 = call "File Dialog"("prompt"="Please Select Folder for Graph Data to be Saved", "default name"=w557) -> ("selected path"=w560:path)  [unwired: 10 in, 3 out]
              n188 = Path To String(path=w560) -> (string=w558:string)
              n189 = Concatenate Strings(w558, w557, ".csv") -> (w561:string)
              n190 = String To Path(string=w561) -> (path=w559:path)
              "to save" <- w559
              n191 = Build Array(w552, w553, w550, w551) -> (w548:dbl[][])
              "Array-to-save" <- w548
              n192 = call-poly <vilib>:"Write Delimited Spreadsheet.vi"("file path (dialog if empty)"=w559, "format (%s)"="%s", "1D data"=string[] ["Time", "Ball Angle", "P Ducer", "PID Output"], "append to file? (new file:F)"=FALSE, "delimiter (\\t)"=w545) -> ("new file path (Not A Path if cancelled)"=w543:path, "error out"=w542:errorcluster)  [unwired: 9 in]
              n193 = call-poly <vilib>:"Write Delimited Spreadsheet.vi"("file path (dialog if empty)"=w543, "format (%.3f)"="%.3f", "2D data"=w548, "append to file? (new file:F)"=TRUE, "error in (no error)"=w542, "transpose? (no:F)"=TRUE, "delimiter (\\t)"=w545) -> ()  [unwired: 7 in, 2 out]
            }
          }
          n194 = property on="Connected" class="Bool (strict)"() -> ("Value"=w223:bool)  [unwired: 2 in, 2 out]
          n195 = call "readVisaMaybe.vi"("Bit in"=64, "error in"=w224, "VISA resource name in"=w226, "VISA connected?"=w223) -> ("String Read"=→"Motor Response":string, "error out"=w221:errorcluster, "VISA resource name out"=w220:refnum<visa-resource-name>)  [unwired: 1 in]
          n196 = event shown="[0] Timeout" {
            selector: _ -> [_ _ _]
            dyn-events: _ -> [_ _ _]
            timeout: w239 -> [_ _ _]
            tunnel: [_ w282 w283] -> w240
            event Timeout {
              n197 = event-data() -> ()  [unwired: 1 in, 3 out]
            }
            event "Set setPoint": Value Change {
              n198 = event-data() -> ("NewVal"=w282:dbl)  [unwired: 1 in, 5 out]
            }
            event "setPoint Dial": Value Change {
              n199 = event-data() -> ("NewVal"=w283:dbl)  [unwired: 1 in, 5 out]
            }
          }
          n200 = event shown="[0] \"Set Angle (º)\": Value Change" {
            selector: _ -> [_ _ _]
            dyn-events: _ -> [_ _ _]
            timeout: w239 -> [_ _ _]
            tunnel: [w284 w285 _] -> _
            event "Set Angle (º)": Value Change {
              n201 = event-data() -> ("NewVal"=w284:dbl)  [unwired: 1 in, 5 out]
            }
            event "Set Angle": Value Change {
              n202 = event-data() -> ("NewVal"=w285:dbl)  [unwired: 1 in, 5 out]
            }
            event Timeout {
              n203 = event-data() -> ()  [unwired: 1 in, 3 out]
            }
          }
          "Set Motor RPM" <- "motor rpm indicator"
          "Motor Signal" <- w255
          "target PID point" <- w241
          "Connected" <- "Connect arduino"
        }
        n204 = while {
          tunnel: [w46] -> w23
          tunnel: w22 -> [w43]
          shift-right: [w72] -> _
          shift-left: _ -> [w71]
          shift-right: [w48] -> _
          shift-left: _ -> [w47]
          stop <- "loop stop 1" stop-if-true
          (unwired) 2
          w53 = 50.0
          # "threshold"
          n205 = property on="Labjack Handle" class="DigNum (strict)"() -> ("Value"=w70:i32)  [unwired: 2 in, 2 out]
          n206 = Get Queue Status(queue=w43, return elements? (F)=TRUE) -> (elements=→"elements":T1[])  [unwired: 1 in, 7 out]
          n207 = Dequeue Element(queue=w43) -> (queue out=w39:refnum<queue>, element=w44:T1, error out=w40:errorcluster)  [unwired: 2 in, 1 out]
          n208 = property on="labjacksModeEnum" class="Enum (strict)"(error in=w40, "Value"=w44) -> ()  [unwired: 1 in, 2 out]
          n209 = case shown="\"Arduino Sensors\"" w44 {
            tunnel: [_ w131 _ w171 _ _] -> w72
            tunnel: w70 -> [_ w133 _ _ _ _]
            tunnel: [_ w132 _ _ _ _] -> _
            tunnel: w39 -> [w112 w125 w147 w169 w181 w196]
            tunnel: [w111 w125 w147 w169 w181 w196] -> w38
            tunnel: "Sensor Loop Rate (ms)" -> [_ _ _ _ _ _]
            tunnel: [w108 w127 w148 w168 w183 w197] -> w48
            tunnel: w71 -> [_ w126 _ _ _ _]
            tunnel: w47 -> [w108 _ _ w168 w184 w197]
            frame "Idle" {
              w109 = T6."Enabled" ("Disabled")
              n210 = property on="Start Sensors" class="Bool"("DisabledEnum"=w109) -> ()  [unwired: 2 in, 2 out]
              n211 = property on="Save Inputs" class="Bool"("DisabledEnum"=w109) -> ()  [unwired: 2 in, 2 out]
              n212 = property on="Load Inputs" class="Bool"("DisabledEnum"=w109) -> ()  [unwired: 2 in, 2 out]
              n213 = property on="Use Dummy Data" class="Bool (strict)"("DisabledEnum"=w109) -> ()  [unwired: 2 in, 2 out]
              n214 = property on="Stop Sensors" class="Bool"("DisabledEnum"=T6."Disabled and Grayed Out" ("Disabled")) -> ()  [unwired: 2 in, 2 out]
              n215 = event shown="[1] \"Load Inputs\": Value Change" {
                selector: _ -> [_ _ _ _]
                dyn-events: _ -> [_ _ _ _]
                timeout: _ -> [_ _ _ _]
                tunnel: w112 -> [w115 w118 w121 w124]
                tunnel: [w114 w117 w120 w123] -> w111
                event "Save Inputs": Value Change {
                  n216 = event-data() -> ()  [unwired: 1 in, 6 out]
                  n217 = Enqueue Element(queue=w115, element=labjacksModeEnum."Idle" ("labjacksModeEnum")) -> (queue out=w114:refnum<queue>)  [unwired: 2 in, 2 out]
                }
                event "Load Inputs": Value Change {
                  n218 = event-data() -> ()  [unwired: 1 in, 6 out]
                  n219 = Enqueue Element(queue=w118, element=labjacksModeEnum."Idle" ("labjacksModeEnum")) -> (queue out=w117:refnum<queue>)  [unwired: 2 in, 2 out]
                }
                event "Start Sensors": Value Change {
                  n220 = event-data() -> ()  [unwired: 1 in, 6 out]
                  n221 = Enqueue Element(queue=w121, element=labjacksModeEnum."Start sensors" ("labjacksModeEnum")) -> (queue out=w120:refnum<queue>)  [unwired: 2 in, 2 out]
                }
                event "Use Dummy Data": Value Change {
                  n222 = event-data() -> ()  [unwired: 1 in, 6 out]
                  n223 = Enqueue Element(queue=w124, element=labjacksModeEnum."Dummy data" ("labjacksModeEnum")) -> (queue out=w123:refnum<queue>)  [unwired: 2 in, 2 out]
                }
              }
            }
            frame "Start sensors" {
              w128 = T6."Disabled and Grayed Out" ("Disabled")
              n224 = event shown="[0] \"Use Avg\": Value Change" {
                selector: _ -> [_ _ _ _]
                dyn-events: _ -> [_ _ _ _]
                timeout: 50 -> [_ _ _ _]
                event "Use Avg": Value Change {
                  n225 = event-data() -> ("NewVal"=w135:bool)  [unwired: 1 in, 5 out]
                  n226 = case shown="True" w135 {
                    frame False {
                    }
                    frame True {
                      n227 = property on="Ducer1" class="Bool (strict)"("Value"=FALSE) -> ()  [unwired: 2 in, 2 out]
                      n228 = property on="Avg Ducers" class="Bool (strict)"("Value"=TRUE) -> ()  [unwired: 2 in, 2 out]
                      n229 = property on="Ducer2" class="Bool (strict)"("Value"=FALSE) -> ()  [unwired: 2 in, 2 out]
                    }
                  }
                }
                event "Use D2": Value Change {
                  n230 = event-data() -> ("NewVal"=w139:bool)  [unwired: 1 in, 5 out]
                  n231 = case shown="True" w139 {
                    frame False {
                    }
                    frame True {
                      n232 = property on="Ducer1" class="Bool (strict)"("Value"=FALSE) -> ()  [unwired: 2 in, 2 out]
                      n233 = property on="Avg Ducers" class="Bool (strict)"("Value"=FALSE) -> ()  [unwired: 2 in, 2 out]
                      n234 = property on="Ducer2" class="Bool (strict)"("Value"=TRUE) -> ()  [unwired: 2 in, 2 out]
                    }
                  }
                }
                event "Use D1": Value Change {
                  n235 = event-data() -> ("NewVal"=w143:bool)  [unwired: 1 in, 5 out]
                  n236 = case shown="True" w143 {
                    frame False {
                    }
                    frame True {
                      n237 = property on="Ducer1" class="Bool (strict)"("Value"=TRUE) -> ()  [unwired: 2 in, 2 out]
                      n238 = property on="Avg Ducers" class="Bool (strict)"("Value"=FALSE) -> ()  [unwired: 2 in, 2 out]
                      n239 = property on="Ducer2" class="Bool (strict)"("Value"=FALSE) -> ()  [unwired: 2 in, 2 out]
                    }
                  }
                }
                event Timeout {
                  n240 = event-data() -> ()  [unwired: 1 in, 3 out]
                }
              }
              n241 = property on="Stop Sensors" class="Bool"("DisabledEnum"=T6."Enabled" ("Disabled")) -> ()  [unwired: 2 in, 2 out]
              n242 = property on="Load Inputs" class="Bool"("DisabledEnum"=w128) -> ()  [unwired: 2 in, 2 out]
              n243 = property on="Save Inputs" class="Bool"("DisabledEnum"=w128) -> ()  [unwired: 2 in, 2 out]
              n244 = property on="Start Sensors" class="Bool"("DisabledEnum"=w128) -> ()  [unwired: 2 in, 2 out]
              n245 = property on="Use Dummy Data" class="Bool (strict)"("DisabledEnum"=w128) -> ()  [unwired: 2 in, 2 out]
              n246 = call "LJM_eReadNames.vi"("Handle In"=w133, "aNames"=string[] ["AIN0", "AIN3", "AIN2_EF_READ_A", "AIN4"], "error in"=w126) -> ("Handle Out"=w132:i32, "aValuesOut"=w127:dbl[], "error out"=w131:errorcluster)  [unwired: 9 in, 1 out]
            }
            frame "Dummy data" {
              w151 = T6."Disabled and Grayed Out" ("Disabled")
              n247 = event shown="[3] Timeout" {
                selector: _ -> [_ _ _ _]
                dyn-events: _ -> [_ _ _ _]
                timeout: 50 -> [_ _ _ _]
                event "Use Avg": Value Change {
                  n248 = event-data() -> ("NewVal"=w156:bool)  [unwired: 1 in, 5 out]
                  n249 = case shown="True" w156 {
                    frame False {
                    }
                    frame True {
                      n250 = property on="Ducer1" class="Bool (strict)"("Value"=FALSE) -> ()  [unwired: 2 in, 2 out]
                      n251 = property on="Avg Ducers" class="Bool (strict)"("Value"=TRUE) -> ()  [unwired: 2 in, 2 out]
                      n252 = property on="Ducer2" class="Bool (strict)"("Value"=FALSE) -> ()  [unwired: 2 in, 2 out]
                    }
                  }
                }
                event "Use D2": Value Change {
                  n253 = event-data() -> ("NewVal"=w160:bool)  [unwired: 1 in, 5 out]
                  n254 = case shown="True" w160 {
                    frame False {
                    }
                    frame True {
                      n255 = property on="Ducer1" class="Bool (strict)"("Value"=FALSE) -> ()  [unwired: 2 in, 2 out]
                      n256 = property on="Avg Ducers" class="Bool (strict)"("Value"=FALSE) -> ()  [unwired: 2 in, 2 out]
                      n257 = property on="Ducer2" class="Bool (strict)"("Value"=TRUE) -> ()  [unwired: 2 in, 2 out]
                    }
                  }
                }
                event "Use D1": Value Change {
                  n258 = event-data() -> ("NewVal"=w164:bool)  [unwired: 1 in, 5 out]
                  n259 = case shown="True" w164 {
                    frame False {
                    }
                    frame True {
                      n260 = property on="Ducer1" class="Bool (strict)"("Value"=TRUE) -> ()  [unwired: 2 in, 2 out]
                      n261 = property on="Avg Ducers" class="Bool (strict)"("Value"=FALSE) -> ()  [unwired: 2 in, 2 out]
                      n262 = property on="Ducer2" class="Bool (strict)"("Value"=FALSE) -> ()  [unwired: 2 in, 2 out]
                    }
                  }
                }
                event Timeout {
                  n263 = event-data() -> ()  [unwired: 1 in, 3 out]
                }
              }
              n264 = property on="Stop Sensors" class="Bool"("DisabledEnum"=T6."Enabled" ("Disabled")) -> ()  [unwired: 2 in, 2 out]
              n265 = property on="Load Inputs" class="Bool"("DisabledEnum"=w151) -> ()  [unwired: 2 in, 2 out]
              n266 = property on="Save Inputs" class="Bool"("DisabledEnum"=w151) -> ()  [unwired: 2 in, 2 out]
              n267 = property on="Use Dummy Data" class="Bool (strict)"("DisabledEnum"=w151) -> ()  [unwired: 2 in, 2 out]
              n268 = property on="Start Sensors" class="Bool"("DisabledEnum"=w151) -> ()  [unwired: 2 in, 2 out]
              n269 = Random Number (0-1)() -> (number: 0 to 1=w152:dbl)
              n270 = Random Number (0-1)() -> (number: 0 to 1=w153:dbl)
              n271 = Random Number (0-1)() -> (number: 0 to 1=w154:dbl)
              n272 = Random Number (0-1)() -> (number: 0 to 1=w155:dbl)
              n273 = Build Array(w155, w154, w153, w152) -> (w148:dbl[])
            }
            frame "Connect to Labjack" {
              n274 = call "LJM_OpenS.vi"() -> ("error out"=w178:errorcluster, "Handle"=w174:i32)  [unwired: 10 in]
              n275 = call "LJM_GetHandleInfo.vi"("error in"=w178, "Handle In"=w174) -> ("error out"=w171:errorcluster, "ConnectionType"=→"ConnectionType":i32, "DeviceType"=→"DeviceType":i32, "Handle Out"=w179:i32, "Port"=→"Port":i32)  [unwired: 2 in, 3 out]
              n276 = call "LJM_eWriteNames.vi"("Handle In"=w179, "aNames"=string[] ["AIN0_RANGE", "AIN3_RANGE", "AIN2_EF_CONFIG_A", "AIN2_EF_INDEX", "AIN4_RANGE"], "aValuesIn"=dbl[] [10.0, 10.0, 0.0, 22.0, 10.0]) -> ("Handle Out"=→"Labjack Handle":i32)  [unwired: 10 in, 2 out]
            }
            frame "Arduino Sensors" {
              n277 = property on="Motor Response" class="Str"() -> ("Value"=w189:string)  [unwired: 2 in, 2 out]
              n278 = local read "arduino read response"() -> (w180:string)
              n279 = Scan From String(format string=w180, input string=w189) -> (error out=w182:errorcluster, output 5=w188:dbl, output 6=w187:dbl, output 7=w186:dbl, output 8=w185:dbl)  [unwired: 14 in, 2 out]
              n280 = case shown="Error .." w182 {
                tunnel: w188 -> [w194 _]
                tunnel: w187 -> [w193 _]
                tunnel: w186 -> [w192 _]
                tunnel: w185 -> [w191 _]
                tunnel: w184 -> [_ w195]
                tunnel: [w190 w195] -> w183
                frame No Error {
                  n281 = Build Array(w194, w193, w192, w191) -> (w190:dbl[])
                }
                frame Error {
                }
              }
            }
            frame "load values" {
            }
          }
          "Labjack error" <- w72
          n282 = Wait Until Next ms Multiple(millisecond multiple="Sensor Loop Rate (ms)") -> (millisecond timer value=w77:u32)
          n283 = Divide(x=w77, y=u32 1000) -> (x/y=→"Time Since Start (s)\n(For Reference Only)":dbl)
          n284 = case shown="False" "Stop Sensors" {
            tunnel: w38 -> [w82 w89]
            tunnel: [w81 w88] -> w37
            frame False {
              n285 = local read "Current Sensor Mode"() -> (w80:T1)
              n286 = Not Equal?(x=w80, y=labjacksModeEnum."Idle" ("labjacksModeEnum")) -> (x != y?=w78:bool)
              n287 = case shown="True" w78 {
                tunnel: w82 -> [w83 w86]
                tunnel: [w83 w85] -> w81
                frame False {
                }
                frame True {
                  n288 = local read "Current Sensor Mode"() -> (w84:T1)
                  n289 = Enqueue Element(queue=w86, element=w84) -> (queue out=w85:refnum<queue>)  [unwired: 2 in, 2 out]
                }
              }
            }
            frame True {
              n290 = Enqueue Element(queue=w89, element=labjacksModeEnum."Idle" ("labjacksModeEnum")) -> (queue out=w88:refnum<queue>)  [unwired: 2 in, 2 out]
            }
          }
          n291 = Array Size(array="Sensor Offsets") -> (size(s)=w69:i32)
          n292 = for {
            N: w69 -> [_]
            tunnel: "Sensor Offsets" -> [w104] mode=indexing
            tunnel: "Sensor K-values" -> [w105] mode=indexing
            tunnel: w48 -> [w107] mode=indexing
            tunnel: [w103] -> w67 mode=indexing
            n293 = Multiply(x=w105, y=w107) -> (x*y=w106:dbl)
            n294 = Add(x=w104, y=w106) -> (x+y=w103:dbl)
          }
          n295 = event shown="[0] Timeout" {
            selector: _ -> [_ _]
            dyn-events: _ -> [_ _]
            timeout: 50 -> [_ _]
            tunnel: [w90 w93] -> w46
            tunnel: w37 -> [w90 w94]
            event Timeout {
              n296 = event-data() -> ()  [unwired: 1 in, 3 out]
            }
            event "Sensor Mode": Value Change {
              n297 = event-data() -> ("NewVal"=w92:enum16{"Fake", "Redboard", "Labjacks"})  [unwired: 1 in, 5 out]
              n298 = case shown="\"Fake\", Default" w92 {
                tunnel: [w95 w96 w97] -> w91
                tunnel: [w95 w96 w97] -> _
                frame "Fake", Default {
                  w95 = labjacksModeEnum."Dummy data" ("labjacksModeEnum")
                }
                frame "Redboard" {
                  w96 = labjacksModeEnum."Arduino Sensors" ("labjacksModeEnum")
                }
                frame "Labjacks" {
                  w97 = labjacksModeEnum."Connect to Labjack" ("labjacksModeEnum")
                }
              }
              n299 = Enqueue Element(queue=w94, element=w91) -> (queue out=w93:refnum<queue>)  [unwired: 2 in, 2 out]
            }
          }
          n300 = Index Array(array=w67, index=T4."Potentiometer" ("labjacksInputs")) -> ()  [unwired: 1 out]
          n301 = Index Array(array=w67, index=T4."Thermocouple" ("labjacksInputs")) -> (element=→"?" →"Stagnation Flow Temp (K)":dbl)
          n302 = Index Array(array=w67, index=T5."Ducer2" ("labjacksInputs")) -> (element=w57:dbl)
          "Pressure Ducer" <- w57
          n303 = Index Array(array=w67, index=T4."Ducer2" ("labjacksInputs")) -> (element=w59:dbl)
          "Pressure Ducer 2" <- w59
          n304 = Subtract(x=w59, y=w57) -> (x-y=w66:dbl)
          n305 = Add(x=w59, y=w57) -> (x+y=w64:dbl)
          n306 = Absolute Value(x=w66) -> (abs(x)=w65:dbl)
          n307 = Divide(x=w64, y=2) -> (x/y=w58:dbl)
          n308 = In Range and Coerce(upper limit=w53, x=w65, lower limit=w53) -> ()  [unwired: 2 out]
          n309 = case shown="False" "Use Avg" {
            tunnel: [w98 w102] -> w63
            tunnel: "Use D2" -> [_ _]
            tunnel: "Use D1" -> [w101 _]
            tunnel: w59 -> [w99 _]
            tunnel: w58 -> [_ w102]
            tunnel: w57 -> [w100 _]
            frame False {
              n310 = Select(t=w99, s=w101, f=w100) -> (s? t:f=w98:dbl)
            }
            frame True {
            }
          }
          "Read Pressure Ducer" <- w63
        }
        n311 = local read "Labjack Handle"() -> (w21:i32)
        n312 = Release Queue(queue=w23) -> ()  [unwired: 2 in, 3 out]
        n313 = Not Equal To 0?(x=w21) -> (x != 0?=w20:bool)
        n314 = case shown="False" w20 {
          tunnel: w21 -> [_ w35]
          frame False {
          }
          frame True {
            n315 = property on="Labjack error" class="Clust (strict)"() -> ("Value"=w34:errorcluster)  [unwired: 2 in, 2 out]
            n316 = call "LJM_Close.vi"("error in"=w34, "Handle"=w35) -> ()  [unwired: 9 in, 1 out]
          }
        }
        n317 = Release Queue(queue=w31) -> ()  [unwired: 2 in, 3 out]
        n318 = call "closeVisaMaybe.vi"("VISA resource name in"=w26, "error in"=w25) -> ("error out"=w24:errorcluster)  [unwired: 9 in]
        "Arduino Error" <- w24
        n319 = Unbundle By Name(w24) -> ("status"=w28:bool)  [unwired: 2 out]
        n320 = Not(x=w28) -> (.not. x?=→"arduino status":bool)
      }
      frame "IdleControllers", Default {
        n321 = property on="Start Program" class="Bool (strict)"() -> ("Value"=w569:bool)  [unwired: 2 in, 2 out]
        n322 = case shown="False" w569 {
          tunnel: w567 -> [w572 w574]
          tunnel: [w571 w573] -> w568
          frame False {
            n323 = Enqueue Element(queue=w572, element=ControllerModeEnum."IdleControllers" ("ControllerModeEnum")) -> (queue out=w571:refnum<queue>)  [unwired: 2 in, 2 out]
          }
          frame True {
            n324 = Enqueue Element(queue=w574, element=ControllerModeEnum."startControllers" ("ControllerModeEnum")) -> (queue out=w573:refnum<queue>)  [unwired: 2 in, 2 out]
          }
        }
      }
    }
    n325 = And(x="Start Program", y="Disconnect") -> (x .and. y?=w16:bool)
  }
